vi "XIS Get Lib Version.vi"(8 "error in (no error)":errorcluster, 10 "bufferSize":i32, 11 "buffer":string) -> (0 "error out":errorcluster, 2 "function return":i32, 3 "buffer out":string)   [LabVIEW 2025, in "VarexWrapper.lvlib"]
doc: "VAREX_API int XIS_GetLibVersion(char *buffer, int bufferSize);"
uses:
  VarexWrapper.lvlib
  VarexWrapper.dll
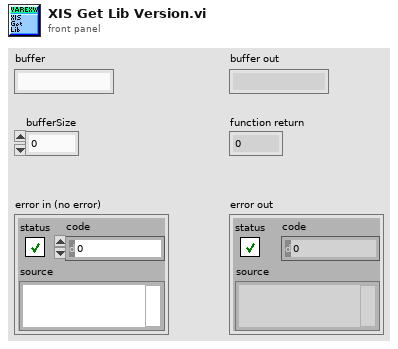
[diagram p1: front panel]
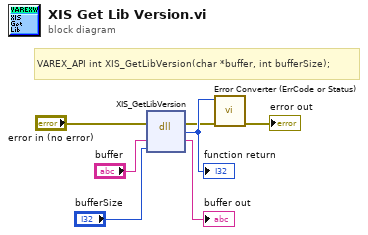
[diagram p0: block diagram]
diagram:
  # "VAREX_API int XIS_GetLibVersion(char *buffer, int bufferSize);"
  n1 = dll-call lib="C:/Users/AriNutpam User/Documents/GitHub/The-Oracle/Image Acquisition/Child Classes/VarexImager/VarexWrapperLvLib/VarexWrapper.*" fn="XIS_GetLibVersion"(error in="error in (no error)", "buffer"="buffer", "bufferSize"="bufferSize") -> (error out=w2:errorcluster, w7:i32, "buffer"=→"buffer out":string)  [unwired: 3 in, 1 out]
  "function return" <- w7
  n2 = call "Error Converter (ErrCode or Status).vi"("error in (no error)"=w2, "error code"=w7) -> ("error out"=→"error out":errorcluster)  [unwired: 9 in]
